vi "RDB Init.vi"(8 "error in":errorcluster, 11 "Compiled.Settings":T5={"Name"="", "RDB Data Receive "=[], "RDB Data Sent"=[], "vclient"=path "", "Network Settings"={"IP adress"="127.0.0.1", "RDB"={"Protocol"=enum."UDP", "Tx Port"=48270, "Rx Port"=10, "Buffer Size"=204800, "Timeout"=10}, "SCP"={"Protocol"=enum."TCP", "Tx Port"=48191, "Rx Port"=48191, "Buffer Size"=204800, "Timeout"=10}}, "SensorInfos"=[], "mmanager"=path "", "Scenario Paths"=[], "Custom SCP Commands"=[], "Timed Loop Settings for TaskControl"={"Period(ms)"=2, "Priority"=100, "Processor"=-2}, "Timed Loop Settings for ModuleManager"={"Period(ms)"=2, "Priority"=100, "Processor"=-2}}) -> (0 "error out":errorcluster, 2 "RDB References":T4, 3 "Settings":T1={"UDP Receiver"=refnum, "UDP Sender"=refnum, "Valid Packet"=FALSE, "TCP"=refnum, "Network Settings"={"IP adress"="127.0.0.1", "RDB"={"Protocol"=enum."UDP", "Tx Port"=48191, "Rx Port"=48191, "Buffer Size"=204800, "Timeout"=10}, "SCP"={"Protocol"=enum."TCP", "Tx Port"=48191, "Rx Port"=48191, "Buffer Size"=204800, "Timeout"=10}}, "vclient"=path "", "paeseHandle"=0, "builderHandle"=0})   [LabVIEW 2023, in "RDB.lvlib"]
uses:
  RDB.lvlib
  Shared/Compiled.Settings.ctl
  System Explorer/RDB Data.ctl
  RDB Player Object.ctl
  Shared/Network Settings.ctl
  Shared/Protocol.ctl
  Shared/SensorInfos.ctl
  Shared/SensorInfo.ctl
  Shared/Sensor Name.ctl
  MM/MM Data.ctl
  MM/MM Objects.ctl
  MM/MM Object.ctl
  Shared/Timedloop Settings.ctl
  RDB References.ctl
  DataContainer/DataContainer.lvclass
  Engine/Type/Settings.ctl
  Shared/Vires VTD Shared.lvlib
  Engine/Vires VTD Engine.lvlib
  MM/MM.lvlib
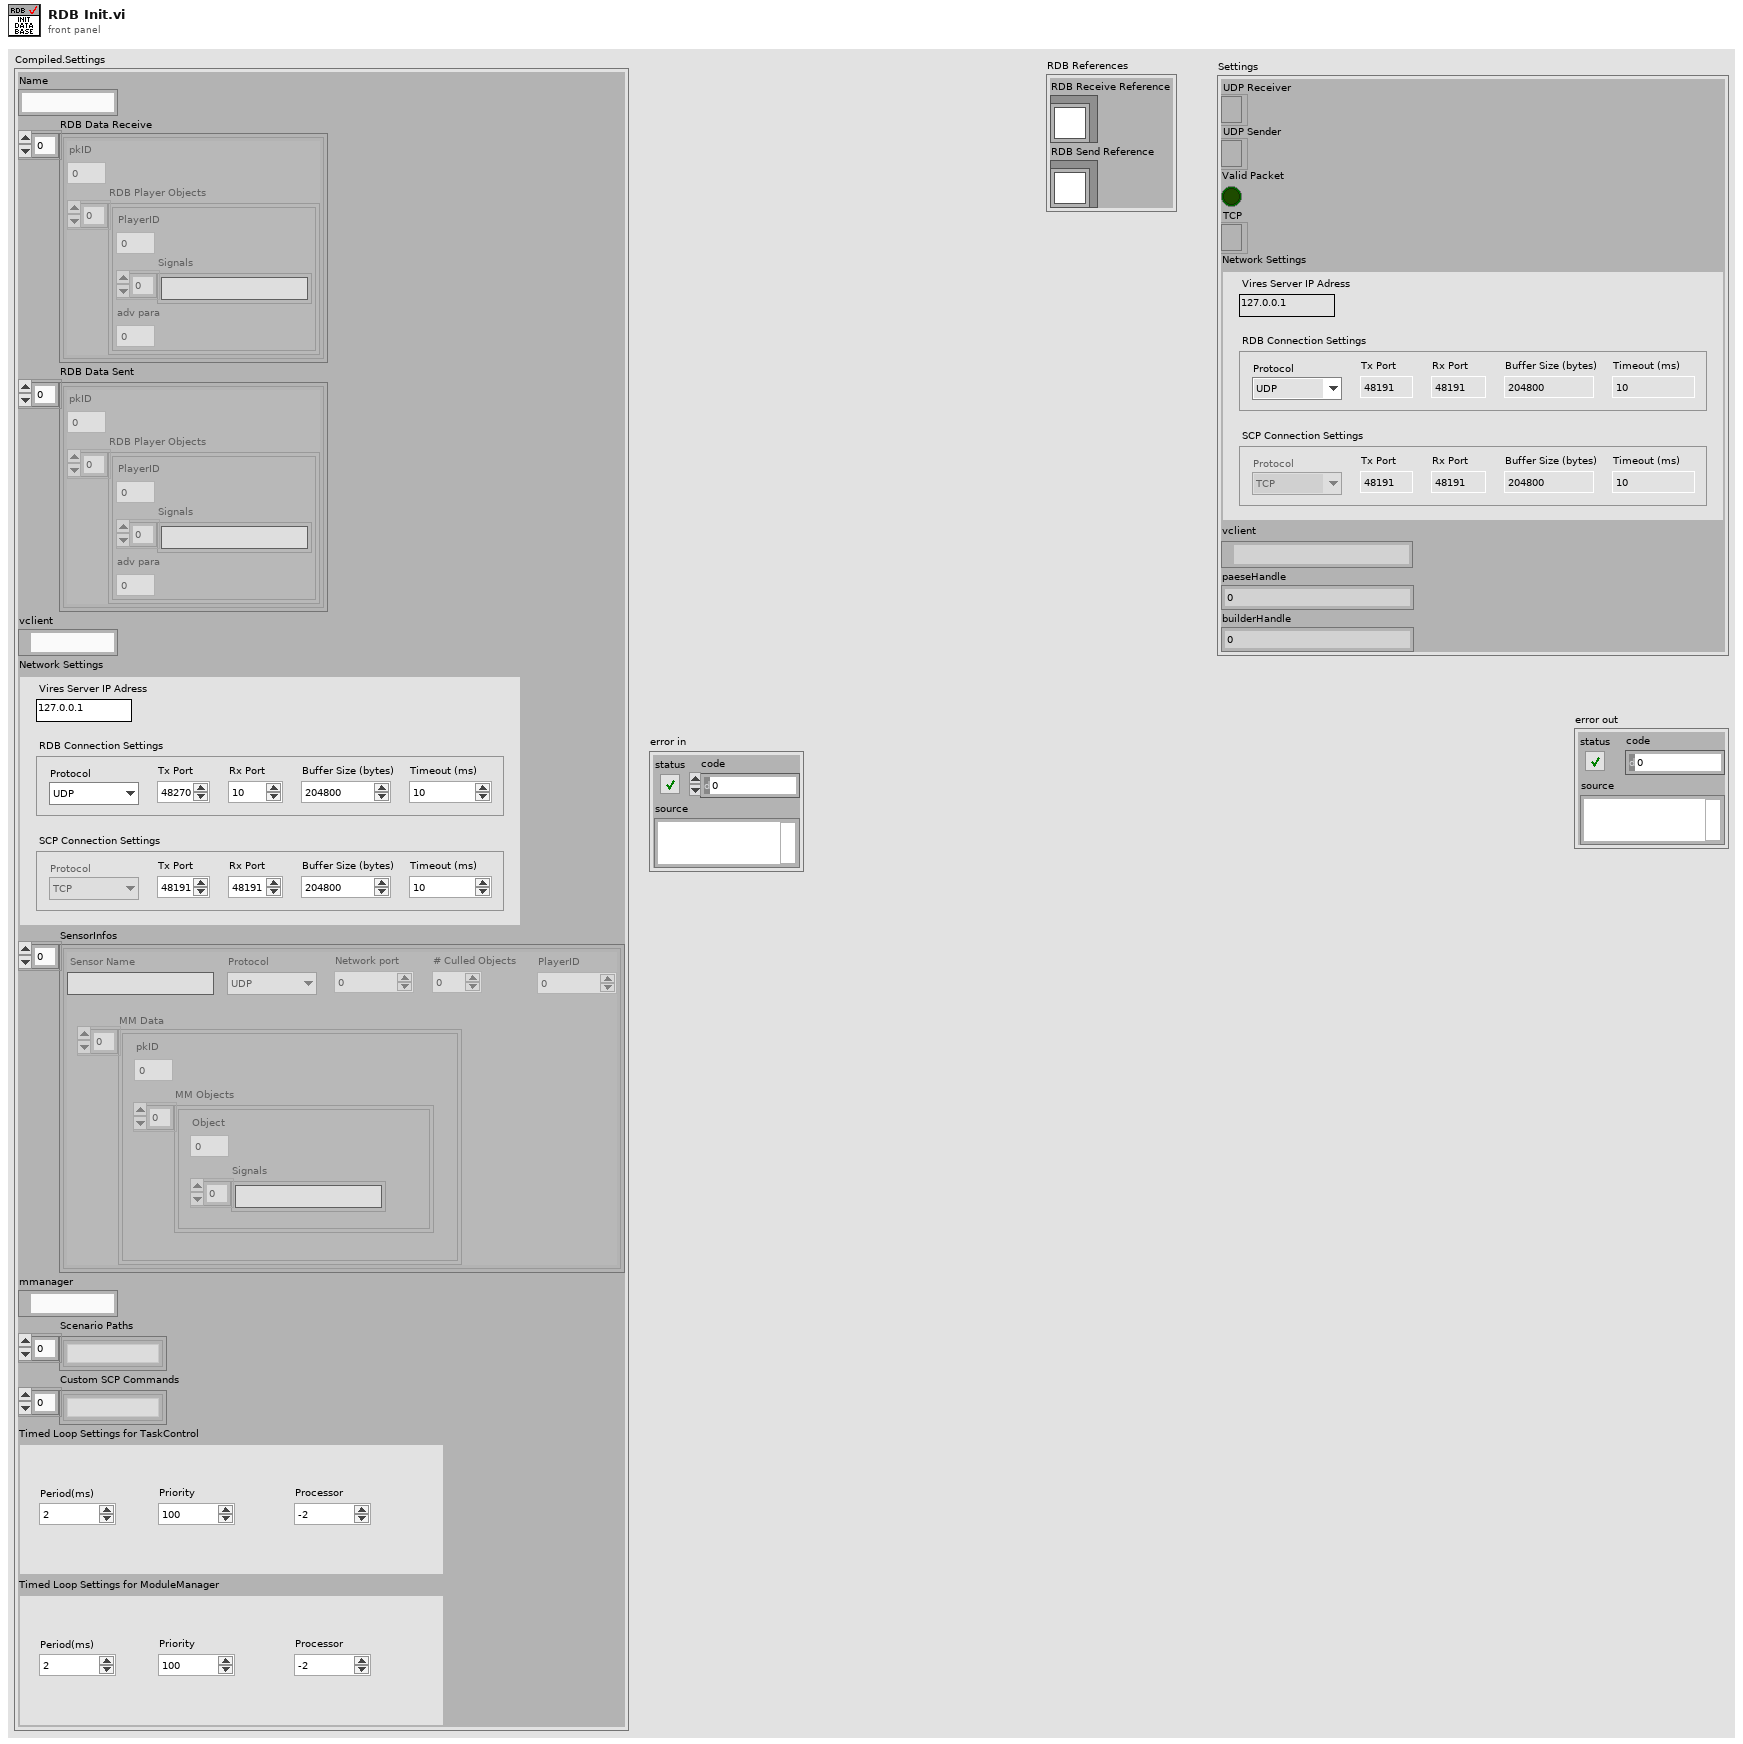
[diagram p1: front panel]
types:
  T1 = typedef "Vires VTD Engine.lvlib/Settings.ctl" = cluster{"UDP Receiver":refnum<k16>, "UDP Sender":refnum<k16>, "Valid Packet":bool, "TCP":refnum<k5>, "Network Settings":T2, "vclient":path, "paeseHandle":u64, "builderHandle":u64}
  T2 = typedef "Vires VTD Shared.lvlib/Network Settings.ctl" = cluster{"IP adress":string, "RDB":cluster{"Protocol":T3, "Tx Port":u16, "Rx Port":u16, "Buffer Size":i32, "Timeout":u16}, "SCP":cluster{"Protocol":T3, "Tx Port":u16, "Rx Port":u16, "Buffer Size":i32, "Timeout":u16}}
  T3 = typedef "Vires VTD Shared.lvlib/Protocol.ctl" = enum16{"UDP", "TCP"}
  T4 = typedef "RDB.lvlib/RDB References.ctl" = cluster{"RDB Receive Reference":refnum<class "DataContainer.lvclass">, "RDB Send Reference":refnum<class "DataContainer.lvclass">}
  T5 = typedef "Vires VTD Shared.lvlib/Compiled.Settings.ctl" = cluster{"Name":string, "RDB Data Receive ":T6, "RDB Data Sent":T6, "vclient":path, "Network Settings":T2, "SensorInfos":T8, "mmanager":path, "Scenario Paths":string[], "Custom SCP Commands":string[], "Timed Loop Settings for TaskControl":T14, "Timed Loop Settings for ModuleManager":T14}
  T6 = typedef "Vires VTD Shared.lvlib/RDB Data.ctl" = cluster{"pkID":i32, "RDB Player Objects":T7[]}[]
  T7 = typedef "RDB.lvlib/RDB Player Object.ctl" = cluster{"PlayerID":i32, "Signals":string[], "adv para":i32}
  T8 = typedef "Vires VTD Shared.lvlib/SensorInfos.ctl" = T9[]
  T9 = typedef "Vires VTD Shared.lvlib/SensorInfo.ctl" = cluster{"Sensor Name":T10, "Protocol":T3, "Network port":i32, "# Culled Objects":i32, "PlayerID":u8, "MM Data":T11}
  T10 = typedef "Vires VTD Shared.lvlib/Sensor Name.ctl" = string
  T11 = typedef "Vires VTD Shared.lvlib/MM Data.ctl" = T12[]
  T12 = typedef "MM.lvlib/MM Objects.ctl" = cluster{"pkID":i32, "MM Objects":T13[]}
  T13 = typedef "MM.lvlib/MM Object.ctl" = cluster{"Object":i32, "Signals":string[]}
  T14 = typedef "Vires VTD Shared.lvlib/Timedloop Settings.ctl" = cluster{"Period(ms)":i64, "Priority":i32, "Processor":i32}
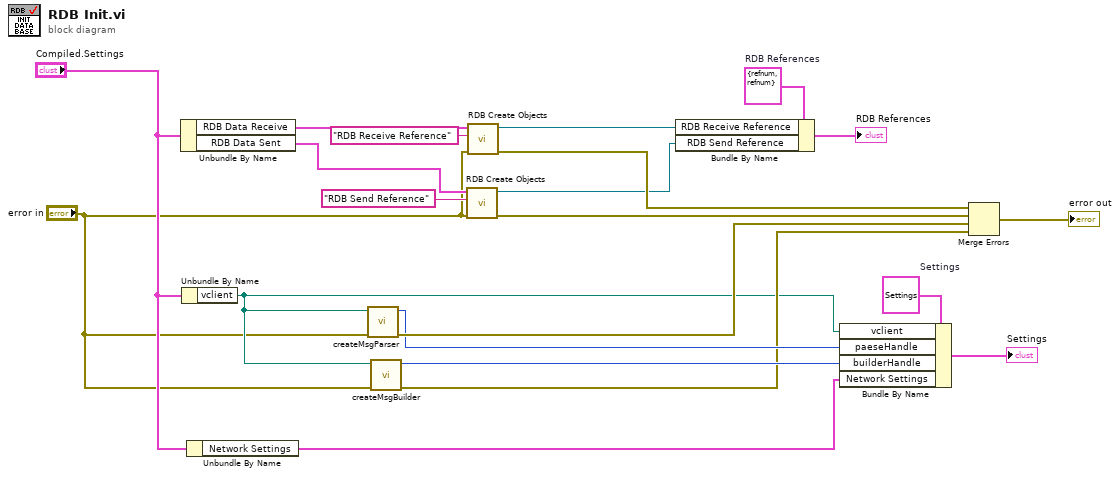
[diagram p0: block diagram]
diagram:
  w14 = T1 {"UDP Receiver"=refnum, "UDP Sender"=refnum, "Valid Packet"=FALSE, "TCP"=refnum, "Network Settings"={"IP adress"="127.0.0.1", "RDB"={"Protocol"=enum."UDP", "Tx Port"=48270, "Rx Port"=10, "Buffer Size"=204800, "Timeout"=10}, "SCP"={"Protocol"=enum."TCP", "Tx Port"=48191, "Rx Port"=48191, "Buffer Size"=204800, "Timeout"=10}}, "vclient"=path "", "paeseHandle"=0, "builderHandle"=0}  # Settings
  w21 = T4 {"RDB Receive Reference"=refnum, "RDB Send Reference"=refnum}  # RDB References
  n1 = Unbundle By Name("Compiled.Settings") -> ("RDB Data Receive"=w19:T6, "RDB Data Sent"=w5:T6)
  n2 = Unbundle By Name("Compiled.Settings") -> ("vclient"=w7:path)
  n3 = Unbundle By Name("Compiled.Settings") -> ("Network Settings"=w9:T2)
  n4 = call "createMsgParser.vi"("error in (no error)"="error in", "path in"=w7) -> ("error out"=w16:errorcluster, "paeseHandle"=w12:u64)  [unwired: 8 in]
  n5 = call "createMsgBuilder.vi"("error in (no error)"="error in", "path in"=w7) -> ("error out"=w8:errorcluster, "builderHandle"=w10:u64)  [unwired: 8 in]
  n6 = call "RDB Create Objects.vi"("error in (no error)"="error in", "Container ID"="RDB Send Reference", "RDB Data Receive"=w5) -> ("error out"=w1:errorcluster, "RDB Reference"=w2:refnum<class "DataContainer.lvclass">)  [unwired: 7 in]
  n7 = call "RDB Create Objects.vi"("error in (no error)"="error in", "Container ID"="RDB Receive Reference", "RDB Data Receive"=w19) -> ("error out"=w18:errorcluster, "RDB Reference"=w20:refnum<class "DataContainer.lvclass">)  [unwired: 7 in]
  n8 = Bundle By Name(cluster=w21, "RDB Receive Reference"=w20, "RDB Send Reference"=w2) -> (→"RDB References":T4)
  n9 = Bundle By Name(cluster=w14, "vclient"=w7, "paeseHandle"=w12, "builderHandle"=w10, "Network Settings"=w9) -> (→"Settings":T1)
  n10 = Merge Errors(w18, w1, w16, w8) -> (→"error out":errorcluster)
